vi "Day 14.vi"() -> ()   [LabVIEW 2021]
uses:
  <vilib>/Utility/file.llb/Read Delimited Spreadsheet (string).vi
panel:
  out "Solution":u64
  in  "Input File":enum32{"example input", "input"}(radio)
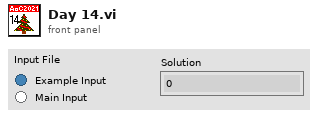
[diagram p1: front panel]
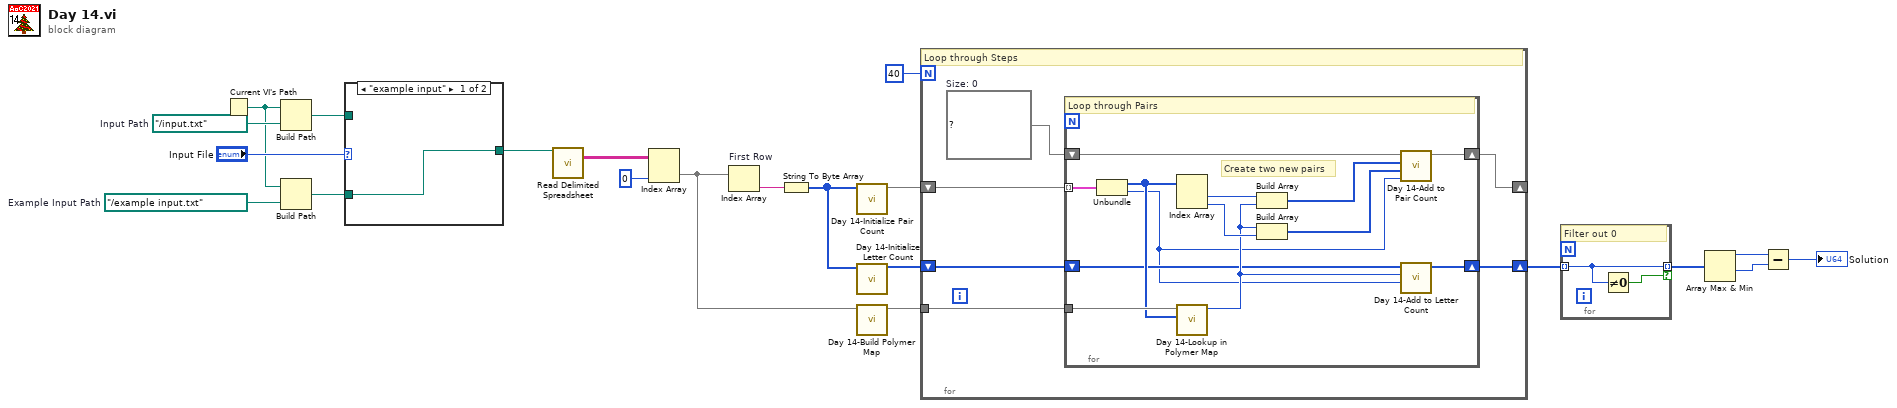
[diagram p0: block diagram]
diagram:
  w20 = path "../example input.txt"  # Example Input Path
  w21 = path "../input.txt"  # Input Path
  n1 = Current VI's Path() -> (path=w15:path)
  n2 = Build Path(base path=w15, name or relative path=w21) -> (appended path=w18:path)
  n3 = Build Path(base path=w15, name or relative path=w20) -> (appended path=w17:path)
  n4 = case shown="\"example input\"" "Input File" {
    tunnel: w18 -> [_ w23]
    tunnel: w17 -> [w22 _]
    tunnel: [w22 w23] -> w16
    frame "example input" {
    }
    frame "input" {
    }
  }
  n5 = call-poly <vilib>:"Read Delimited Spreadsheet.vi"("file path (dialog if empty)"=w16) -> ("all rows"=w14:string[][])  [unwired: 9 in, 5 out]
  n6 = Index Array(array=w14, index (col)=0 ("disabled index (col)")) -> (element=w12:string[])  [unwired: 1 in]
  n7 = Index Array "First Row"(array=w12) -> (element=w6:string)  [unwired: 1 in]
  n8 = String To Byte Array(string=w6) -> (unsigned byte array=w3:u8[])
  n9 = call "Day 14-Initialize Pair Count.vi"("Initial Letters"=w3) -> ("Map"=w5:map{u8[], u64})  [unwired: 10 in]
  n10 = call "Day 14-Initialize Letter Count.vi"("Initial Letters"=w3) -> ("Count Array"=w4:u64[])  [unwired: 10 in]
  n11 = call "Day 14-Build Polymer Map.vi"("Polymer Input"=w12) -> ("Polymer Template Map"=w11:map{string, string})  [unwired: 10 in]
  n12 = for {
    N: 40 -> [_]
    tunnel: w11 -> [w29]
    shift-right: [w27] -> _
    shift-left: w5 -> [w28]
    shift-right: [w25] -> w2
    shift-left: w4 -> [w26]
    w24 = map{u8[], u64} {}  # Size: 0
    # "Loop through Steps"
    n13 = for {
      tunnel: w28 -> [w42] mode=indexing
      tunnel: w29 -> [w35]
      shift-right: [w40] -> w27
      shift-left: w24 -> [w41]
      shift-right: [w37] -> w25
      shift-left: w26 -> [w31]
      # "Create two new pairs"
      # "Loop through Pairs"
      n14 = Unbundle(w42) -> (w34:u8[], w30:u64)
      n15 = Index Array(array=w34) -> (element #1=w39:u8, element #2=w38:u8)  [unwired: 2 in]
      n16 = call "Day 14-Lookup in Polymer Map.vi"("Pair"=w34, "Polymer Template Map"=w35) -> ("New Entry"=w36:u8)  [unwired: 9 in]
      n17 = Build Array(w39, w36) -> (w33:u8[])
      n18 = Build Array(w36, w38) -> (w32:u8[])
      n19 = call "Day 14-Add to Pair Count.vi"("Count"=w30, "Pair 2"=w32, "Pair 1"=w33, "Count in"=w41) -> ("Count out"=w40:map{u8[], u64})  [unwired: 7 in]
      n20 = call "Day 14-Add to Letter Count.vi"("Count"=w30, "New Entry"=w36, "Count Array in"=w31) -> ("Count Array out"=w37:u64[])  [unwired: 8 in]
    }
  }
  n21 = for {
    tunnel: w2 -> [w44] mode=indexing
    tunnel: [w44] -> w1 mode=indexing if=w43
    # "Filter out 0"
    n22 = Not Equal To 0?(x=w44) -> (x != 0?=w43:bool)
  }
  n23 = Array Max & Min(array=w1) -> (max value=w9:u64, min value=w7:u64)  [unwired: 2 out]
  n24 = Subtract(x=w9, y=w7) -> (x-y=→"Solution":u64)
